vi "New Data Item Filter.vi"   [LabVIEW 2018, in "GLog.lvlib" / "Data Item.lvclass"]
doc: "Creates a new Filter which matches log calls based on the contents of the data field. Matches are based on the names of data items, not the values.\nExample:\nIf a log call has data \"{custom: 42069}\" and the filter is setup with data item \"custom\", it will match. If the filter is setup with data item \"42069\" it will not match."
uses:
  Data Item.lvclass
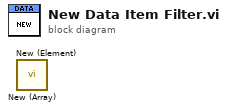
[diagram p0: block diagram]
diagram:
  n1 = call "New (Array).vi"() -> ()  [unwired: 10 in, 2 out]
  n2 = call "New (Element).vi"() -> ()  [unwired: 10 in, 2 out]
